vi "NR wait Call Connection.vi"(8 "error in (no error)":errorcluster caption="에러 입력(에러 없음)", 10 "Waiting Time":i32, 11 "Instrument Manager 입력":refnum<class "Instrument Manager.lvclass">) -> (0 "error out":errorcluster caption="에러 출력", 2 "Connected?":bool, 3 "Instrument Manager 출력":refnum<class "Instrument Manager.lvclass">)   [LabVIEW 2023, in "Instrument Manager.lvclass"]
uses:
  Instrument Manager.lvclass
  Instrument Manager.lvclass/Instrument Manager.ctl
  Module/ANRITSU Call Box/Type Definition/Call Processing Status Enum.ctl
  9bf643c0-3077-4f83-81e7-953a0e6db1c7.vi
  Module/ANRITSU Call Box/Interface Class/Anritsu Call Box.lvclass
  Module/ANRITSU Call Box/ANRITSU Call Box.lvlib
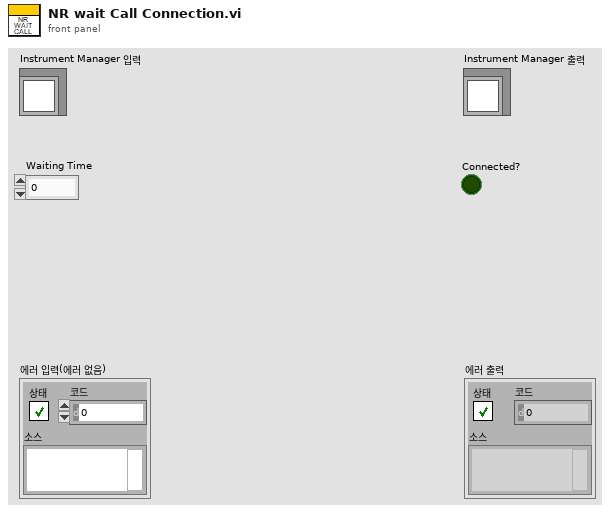
[diagram p1: front panel]
types:
  T1 = typedef "ANRITSU Call Box.lvlib/Call Processing Status Enum.ctl" = enum16{"Off", "Idle", "Idle (Regist)", "Registration", "UE Origination", "NW Origination", "Connected", "SCG Adding", "Connected (NSA)", "SCG Release", "Undefined1", "Undefined2", "Undefined3", "Handover", "NW Release", "UE Release", "Detach", "Setup", "Redirection"}
  T2 = cluster{"Anritsu Call Box":refnum<class "Anritsu Call Box.lvclass">, "Spectrum Analyzer":refnum<class "Interface_Spectrum.lvclass">, "RF Switch Box":refnum<class "RF Filter Box.lvclass">, "Turn Table":refnum<class "Interface - Turn Table.lvclass">, "Mast":refnum<class "Interface - Mast.lvclass">, "3D Controller":refnum<class "Interface_3D Controller.lvclass">}
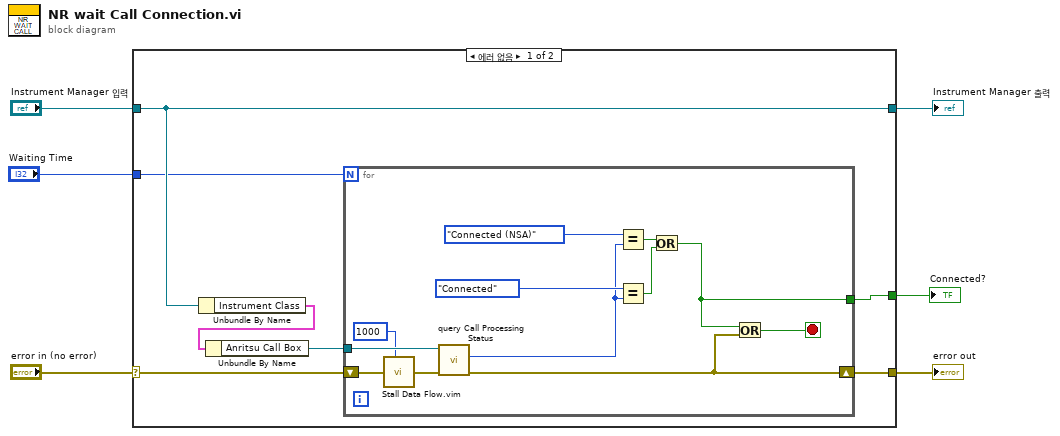
[diagram p0: block diagram]
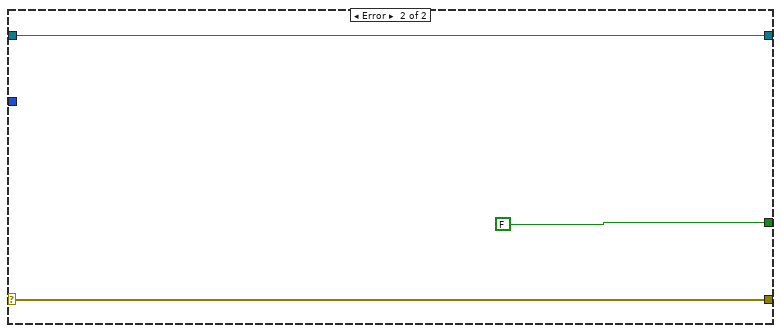
[diagram p2: hidden frame]
diagram:
  n1 = case shown="에러 없음" "error in (no error)" {
    selector: "error in (no error)" -> [w8 w28]
    tunnel: [w9 w28] -> w5
    tunnel: [w13 w27] -> w3
    tunnel: "Instrument Manager 입력" -> [w13 w27]
    tunnel: "Waiting Time" -> [w12 _]
    tunnel: [w7 FALSE] -> w1
    frame No Error {
      n2 = Unbundle By Name(w13) -> ("Instrument Class"=w11:T2)
      n3 = Unbundle By Name(w11) -> ("Anritsu Call Box"=w10:refnum<class "Anritsu Call Box.lvclass">)
      n4 = for {
        N: w12 -> [_]
        tunnel: w10 -> [w24]
        shift-right: [w23] -> w9
        shift-left: w8 -> [w21]
        tunnel: [w14] -> w7
        stop <- w22 stop-if-true
        n5 = call "Stall Data Flow.vim"("value in"=w21, "milliseconds to wait"=u32 1000) -> ("value out"=w20:errorcluster)  [unwired: 1 out]
        n6 = call-dynamic "query Call Processing Status.vi"("error in (no error)"=w20, "Anritsu Call Box in"=w24) -> ("error out"=w23:errorcluster, "Call Processing Status"=w16:T1)  [unwired: 7 in, 1 out]
        n7 = Equal?(x=Call_Processing_Status_Enum."Connected (NSA)" ("Call Processing Status"), y=w16) -> (x = y?=w17:bool)
        n8 = Equal?(x=Call_Processing_Status_Enum."Connected" ("Call Processing Status"), y=w16) -> (x = y?=w15:bool)
        n9 = Or(x=w17, y=w15) -> (x .or. y?=w14:bool)
        n10 = Or(x=w14, y=w23) -> (x .or. y?=w22:bool)
      }
    }
    frame Error {
    }
  }
  "error out" <- w5
  "Instrument Manager 출력" <- w3
  "Connected?" <- w1
